vi "strings to base format.vi"(8 "error in":errorcluster, 11 "1.0.0":T1) -> (0 "error out":errorcluster, 3 "format":T5)   [LabVIEW 2014, in "NISE_CEF_TreeSerializer.lvlib"]
doc: "Converts the set of flattened instance data into the <b>base file format</b> and sets the version number. For version 1.0.0, the format is JSON."
uses:
  NISE_CEF_TreeSerializer.lvlib
  base file format.ctl
  flat hierarchy.ctl
  full hierarchy.ctl
  hierarchy element.ctl
  instance data.ctl
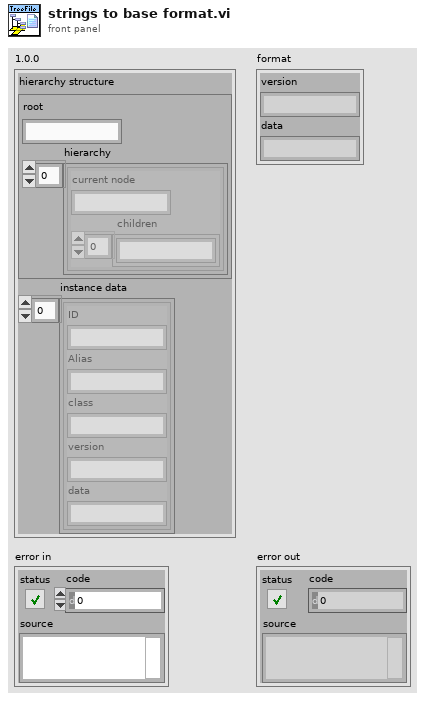
[diagram p1: front panel]
types:
  T1 = typedef "NISE_CEF_TreeSerializer.lvlib/flat hierarchy.ctl" = cluster{"hierarchy structure":T2, "instance data":T4[]}
  T2 = typedef "NISE_CEF_TreeSerializer.lvlib/full hierarchy.ctl" = cluster{"root":string, "hierarchy":T3[]}
  T3 = typedef "NISE_CEF_TreeSerializer.lvlib/hierarchy element.ctl" = cluster{"current node":string, "children":string[]}
  T4 = typedef "NISE_CEF_TreeSerializer.lvlib/instance data.ctl" = cluster{"ID":string, "Alias":string, "class":string, "version":string, "data":string}
  T5 = typedef "NISE_CEF_TreeSerializer.lvlib/base file format.ctl" = cluster{"version":string, "data":string}
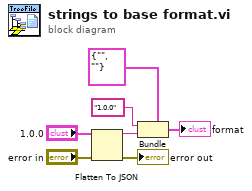
[diagram p0: block diagram]
diagram:
  n1 = Flatten To JSON(anything="1.0.0", error in (no error)="error in") -> (JSON string=w3:string, 11:→"error out":errorcluster)  [unwired: 1 in]
  n2 = Bundle(cluster=T5 {"version"="", "data"=""} ("format"), "version"="1.0.0", "data"=w3) -> (→"format":T5)
